vi "ReadHTTPHeader.vi"(8 "error in (no error)":errorcluster, 10 "timeout ms (25000)":i32=25000, 11 "WebSocket Connection in":refnum<k5>) -> (0 "error out":errorcluster, 2 "HTTP Header":string, 3 "WebSocket Connection out":refnum<k5>)   [LabVIEW 2021, in "LV WebSockets.lvlib"]
doc: "WebSockets 1.6.0.22\nSam Sharp - MediaMongrels Ltd\nCopyright (c) 2016, MediaMongrels Ltd"
uses:
  LV WebSockets.lvlib
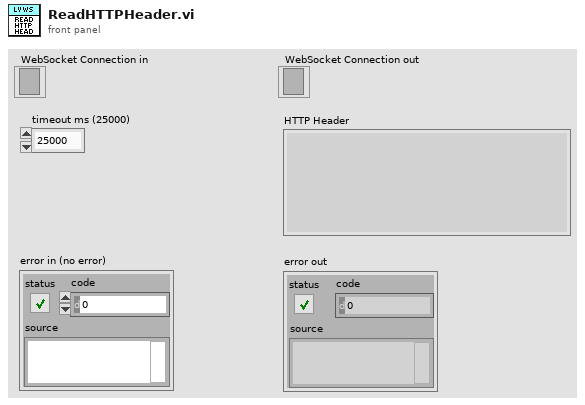
[diagram p1: front panel]
types:
  T1 = enum16{"Standard", "Buffered", "CRLF", "Immediate"}
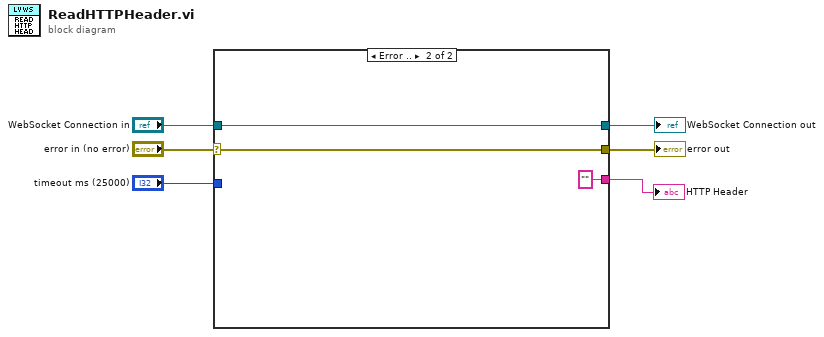
[diagram p0: block diagram]
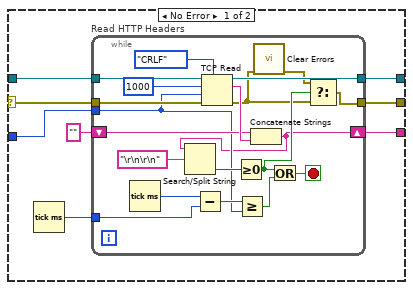
[diagram p2: hidden frame]
diagram:
  n1 = case shown="Error .." "error in (no error)" {
    selector: "error in (no error)" -> [w11 w37]
    tunnel: [w12 w37] -> w6
    tunnel: "timeout ms (25000)" -> [w10 _]
    tunnel: "WebSocket Connection in" -> [w9 w36]
    tunnel: [w8 w36] -> w2
    tunnel: [w7 ""] -> w1
    frame No Error {
      n2 = Tick Count (ms)() -> (millisecond timer value=w14:u32)
      n3 = while "Read HTTP Headers" {
        tunnel: w9 -> [w34]
        tunnel: [w33] -> w8
        shift-right: [w15] -> w7
        shift-left: "" -> [w29]
        tunnel: w10 -> [w22]
        tunnel: [w16] -> w12
        tunnel: w11 -> [w30]
        tunnel: w14 -> [w23]
        stop <- w28 stop-if-true
        n4 = Tick Count (ms)() -> (millisecond timer value=w24:u32)
        n5 = Subtract(x=w24, y=w23) -> (x-y=w26:u32)
        n6 = TCP Read(connection ID=w34, bytes to read=1000, error in (no error)=w30, 7:T1."CRLF" ("mode (standard)"), 9:w22) -> (connection ID out=w33:refnum<k5>, data out=w31:string, error out=w18:errorcluster)
        n7 = Greater Or Equal?(x=w26, y=w22) -> (x >= y?=w25:bool)
        n8 = Concatenate Strings(w29, w31) -> (w15:string)
        n9 = Search/Split String(string=w15, search string/char (-)="\r\n\r\n") -> (offset of match=w27:i32)  [unwired: 1 in, 2 out]
        n10 = Greater Or Equal To 0?(x=w27) -> (x >= 0?=w19:bool)
        n11 = call <vilib>:"Clear Errors.vi"("error in (no error)"=w18) -> ("error out"=w17:errorcluster)  [unwired: 5 in, 1 out]
        n12 = Or(x=w19, y=w25) -> (x .or. y?=w28:bool)
        n13 = Select(t=w17, s=w19, f=w18) -> (s? t:f=w16:errorcluster)
      }
    }
    frame Error {
    }
  }
  "error out" <- w6
  "WebSocket Connection out" <- w2
  "HTTP Header" <- w1
